vi "EJERCICIO _5_BUSQUEDA_ARREGLO_WHILE.vi"() -> ()   [LabVIEW 2026]
panel:
  out "VALOR ENCONTRADO":bool
  in  "VALOR A BUSCAR":dbl
  in  "VALORES":dbl[](array[numeric])
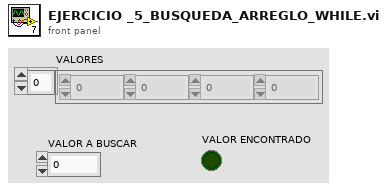
[diagram p1: front panel]
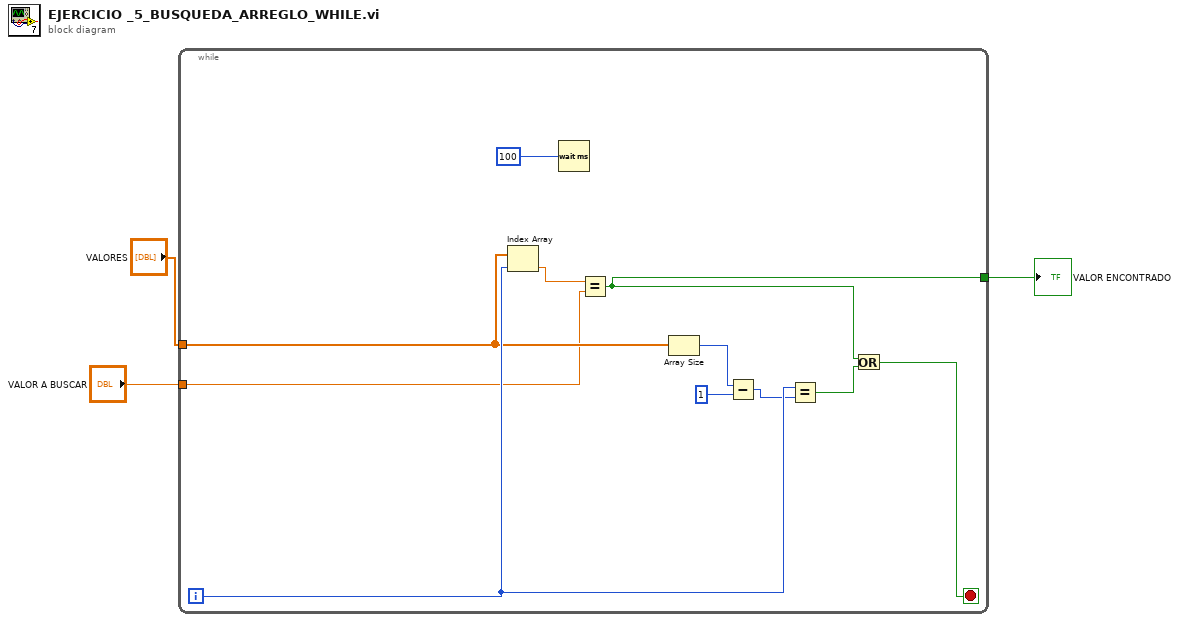
[diagram p0: block diagram]
diagram:
  n1 = while {
    tunnel: "VALORES" -> [w6]
    tunnel: "VALOR A BUSCAR" -> [w5]
    tunnel: [w4] -> w1
    i -> [w10]
    stop <- w7 stop-if-true
    n2 = Index Array(array=w6, index=w10) -> (element=w14:dbl)
    n3 = Wait (ms)(milliseconds to wait=100) -> ()  [unwired: 1 out]
    n4 = Equal?(x=w14, y=w5) -> (x = y?=w4:bool)
    n5 = Array Size(array=w6) -> (size(s)=w12:i32)
    n6 = Subtract(x=w12, y=1) -> (x-y=w9:i32)
    n7 = Equal?(x=w10, y=w9) -> (x = y?=w8:bool)
    n8 = Or(x=w4, y=w8) -> (x .or. y?=w7:bool)
  }
  "VALOR ENCONTRADO" <- w1
